vi "Convert Error.vi"(6 "return type":i32, 8 "error in (no error)":errorcluster) -> (0 "error out":errorcluster)   [LabVIEW 2021, in "Iceoryx.lvlib"]
uses:
  Iceoryx.lvlib
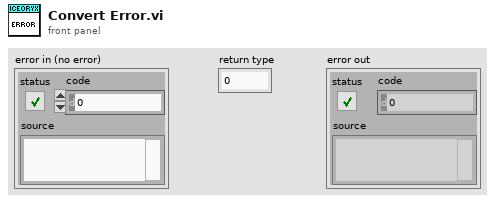
[diagram p1: front panel]
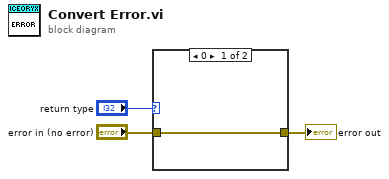
[diagram p0: block diagram]
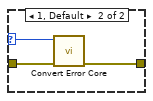
[diagram p2: hidden frame]
diagram:
  n1 = case shown="0" "return type" {
    selector: "return type" -> [_ w7]
    tunnel: "error in (no error)" -> [w4 w6]
    tunnel: [w4 w5] -> w1
    frame 0 {
    }
    frame 1, Default {
      n2 = call "Convert Error Core.vi"("error in (no error)"=w6, "return type"=w7) -> ("error out"=w5:errorcluster)  [unwired: 9 in]
    }
  }
  "error out" <- w1
